vi "SlewRateLimiter_NewInitialZero.vi"(8 "Time":dbl=-1.0 format="%33.4f", 10 "NegativeRateLimit":dbl=1.0, 11 "PositiveRateLimit":dbl) -> (3 "out SLEW_RATE_LIMITER":T1 {"NegativeRateLimit" format="%13.5p"; "PrevTime" format="%30.5p"; "PrevValue" format="%13.5p"; "PositiveRateLimit" format="%13.5p"})   [LabVIEW 2019, in "Trajectory_Library.lvlib"]
doc: "Creates a new SlewRateLimiter data cluster with the given rate limit. The initial value is set to zero.\n\nThis set of functions limits the rate of change of an input value. Useful for implementing voltage, setpoint, and/or output ramps. A slew-rate limit is most appropriate when the quantity being controlled is a velocity or a voltage; when controlling a position, consider using a postion control algoritmn or trapezoid profile instead.\n\nInputs:\n - PositiveRateLimit -- The positive rate-of-change limit, in units per second. \n The value is expected to be >= 0.\n - NegativeRateLimit -- The negative rate-of-change limit, in units per second.\n The value is expected to be <= 0. If the value is not wired or is > 0 then\n the PositiveRateLimit * -1 is used. \n \nOutputs:\n - out Slew Rate Limiter -- The initialized Slew Rate Limiter data cluster"
uses:
  Trajectory_Library.lvlib
  TypeDef/SLEW_RATE_LIMITER.ctl
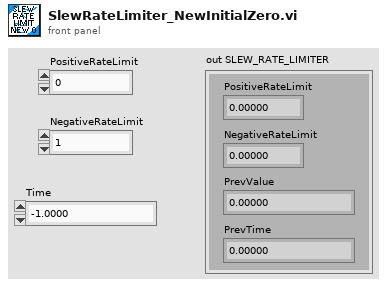
[diagram p1: front panel]
types:
  T1 = typedef "Trajectory_Library.lvlib/SLEW_RATE_LIMITER.ctl" = cluster{"PositiveRateLimit":dbl, "PrevValue":dbl, "PrevTime":dbl, "NegativeRateLimit":dbl}
  T2 = typedef "WPILib_Math.lvlib/SLEW_RATE_LIMITER.ctl" = cluster{"PositiveRateLimit":dbl, "PrevValue":dbl, "PrevTime":dbl, "NegativeRateLimit":dbl}
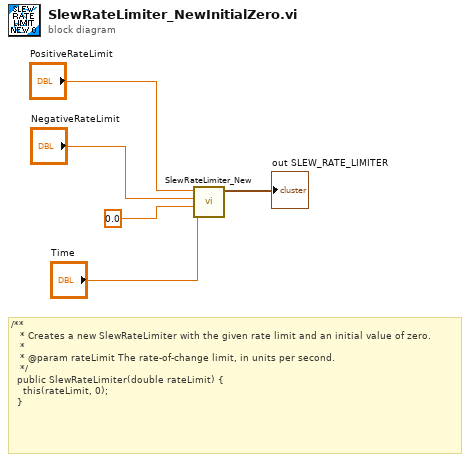
[diagram p0: block diagram]
diagram:
  # "/**\n   * Creates a new SlewRateLimiter with the given rate limit and an initial value of zero.\n   *\n   * @param rateLimit The rate-of-change limit, in units per second.\n   */\n  public SlewRateLimiter(double rateLimit) {\n    this(rateLimit, 0);\n  }"
  n1 = call "SlewRateLimiter_New.vi"("Time"="Time", "InitialValue"=0.0, "NegativeRateLimit"="NegativeRateLimit", "PositiveRateLimit"="PositiveRateLimit") -> ("out SLEW_RATE_LIMITER"=→"out SLEW_RATE_LIMITER":T2)  [unwired: 7 in]
